vi "PicoScope4000Open.vi"(1 "Serial Number":string, 2 "Mode":u16(ring) items=["Dialog On Error", "no dialog - CloseUnit and Stop", "no dialog - Continue", "no dialog - Stop"], 5 "Use Serial Number":bool, 11 "error in (no error)":errorcluster) -> (4 "handle":i16, 12 "Max ADC value":i16, 14 "Unit Info":T1, 15 "error out":errorcluster)   [LabVIEW 2010]
doc: "This VI opens a PicoScope 4000 series and returns a handle to the device."
uses:
  ps4000.dll
panel:
  out "Pico 4000 Units":string
  out "serialLth":i16
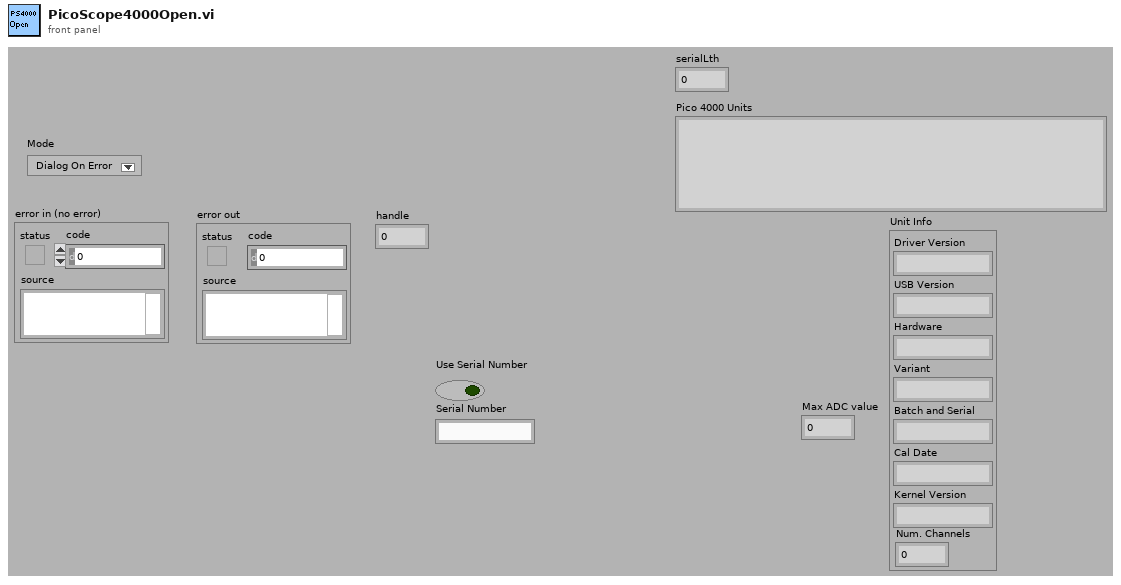
[diagram p1: front panel]
types:
  T1 = cluster{"Driver Version":string, "USB Version":string, "Hardware":string, "Variant":string, "Batch and Serial":string, "Cal Date":string, "Kernel Version":string, "Num. Channels":i16}
  T2 = cluster{"status":bool, "code":u32, "source":string}
  T3 = cluster{"Driver Version":string, "USB Version":string, "Hardware":string, "Variant":string, "Batch and Serial":string, "Cal Date":string, "Kernel Version":string}
  T4 = cluster{"Driver Version":string, "USB Version":string, "Hardware":string, "Variant":string, "Batch and Serial":string, "Cal Date":string, "Kernel Version":string, i16}
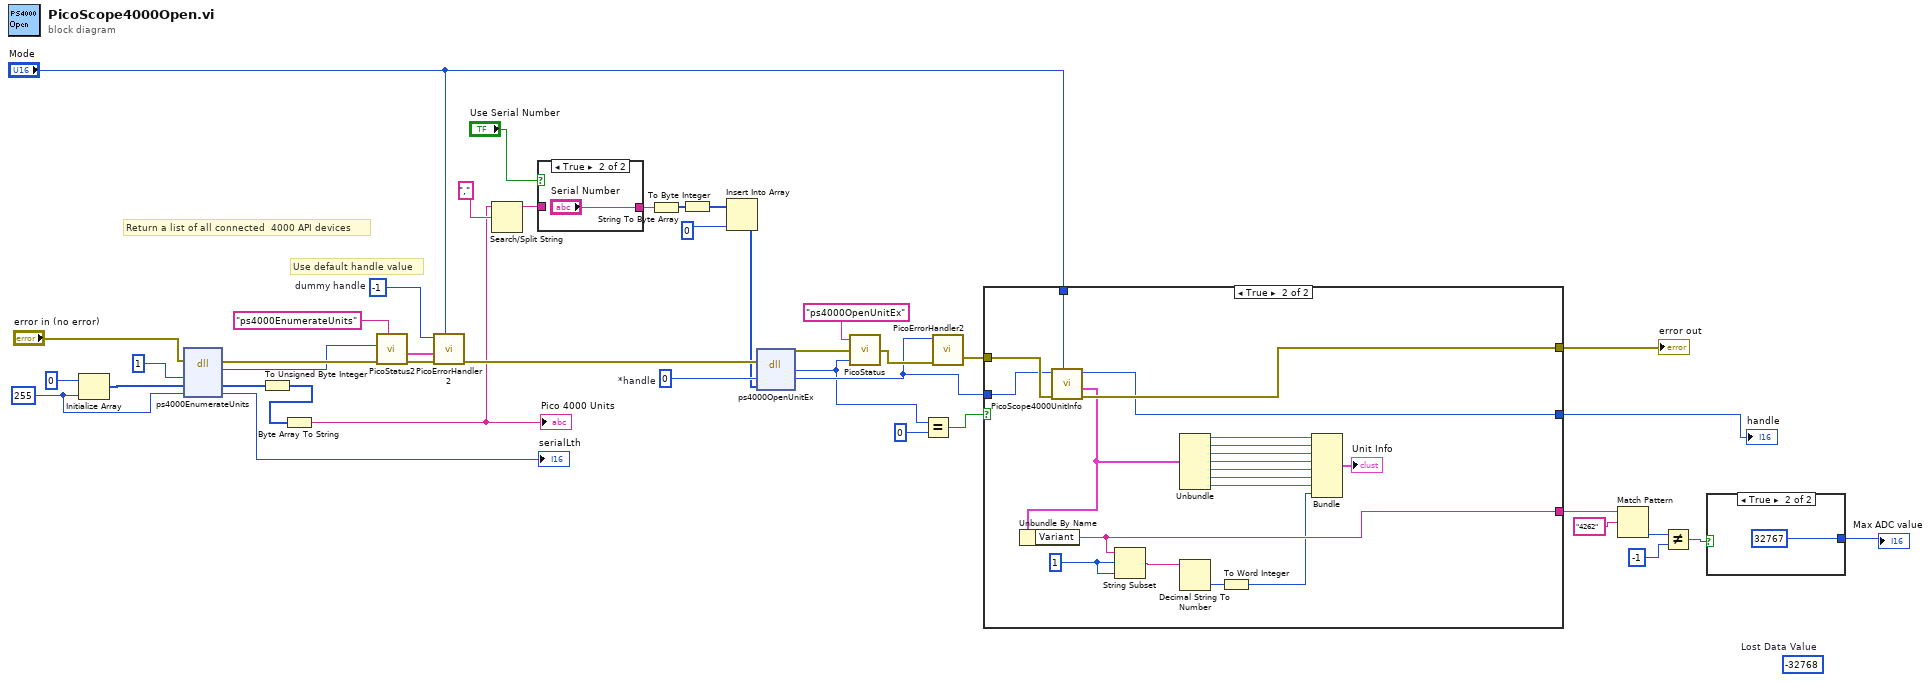
[diagram p0: block diagram]
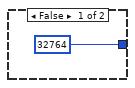
[diagram p3: hidden frame]
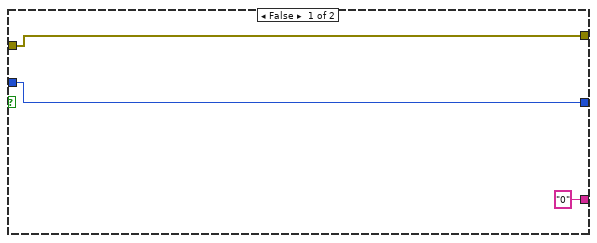
[diagram p4: hidden frame]
diagram:
  w17 = i16 -1  # dummy handle
  w20 = i16 255 ("dimension size")
  (unwired) i16 -32768  # Lost Data Value
  w33 = i16 0  # *handle
  # "Use default handle value"
  # "Return a list of all connected  4000 API devices"
  n1 = Initialize Array(i8 0 ("U8"), w20) -> (w22:i8[])
  n2 = dll-call lib="ps4000.dll" fn="ps4000EnumerateUnits"(error in="error in (no error)", "count"=i16 1, "serials"=w22, "serialLth"=w20) -> (error out=w5:errorcluster, "PICO_STATUS"=w4:u32, "serials"=w18:i8[], "serialLth"=→"serialLth":i16)  [unwired: 3 in, 1 out]
  n3 = To Unsigned Byte Integer(number=w18) -> (unsigned 8bit integer=w19:u8[])
  n4 = Byte Array To String(unsigned byte array=w19) -> (string=w9:string)
  "Pico 4000 Units" <- w9
  n5 = call "PicoStatus2.vi"("PICO source"="ps4000EnumerateUnits" ("source"), "Error in"=w5, "PICO STATUS"=w4) -> ("error out"=w7:errorcluster, "PICO_STATUS out"=w6:T2)  [unwired: 5 in]
  n6 = call "PicoErrorHandler2.vi"("Mode"="Mode", "error in (no error)"=w7, "PICO_STATUS in"=w6, "handle In"=w17) -> ("error out"=w32:errorcluster)  [unwired: 7 in]
  n7 = Search/Split String(string=w9, search string/char (-)=",") -> (substring before match=w15:string)  [unwired: 1 in, 2 out]
  n8 = case shown="True" "Use Serial Number" {
    tunnel: w15 -> [w43 _]
    tunnel: [w43 "Serial Number"] -> w11
    frame False {
    }
    frame True {
    }
  }
  n9 = String To Byte Array(string=w11) -> (unsigned byte array=w13:u8[])
  n10 = To Byte Integer(number=w13) -> (8bit integer=w14:i8[])
  n11 = Insert Into Array(array=w14, new element=i8 0 ("new element/subarray")) -> (w10:i8[])  [unwired: 1 in]
  n12 = dll-call lib="ps4000.dll" fn="ps4000OpenUnitEx"(error in=w32, "handle"=w33, "serial"=w10) -> (error out=w31:errorcluster, "PICO_STATUS"=w28:u32, "handle"=w29:i16)  [unwired: 3 in, 1 out]
  n13 = call "PicoStatus.vi"("PICO STATUS"=w28, "error in"=w31, "source"="ps4000OpenUnitEx") -> ("error out"=w39:errorcluster)
  n14 = Equal?(x=w28, y=i16 0) -> (x = y?=w42:bool)
  n15 = call "PicoErrorHandler2.vi"("error in (no error)"=w39, "handle In"=w29) -> ("error out"=w30:errorcluster)  [unwired: 9 in]
  n16 = case shown="True" w42 {
    tunnel: w29 -> [w47 w55]
    tunnel: [w47 w57] -> w25
    tunnel: [w46 w59] -> w1
    tunnel: w30 -> [w46 w56]
    tunnel: ["0" ("Variant") w50] -> w38
    tunnel: "Mode" -> [_ w48]
    frame False {
    }
    frame True {
      w51 = 1 ("offset (0)")
      n17 = call "PicoScope4000UnitInfo.vi"("Mode"=w48, "error in (no error)"=w56, "handle in"=w55) -> ("error out"=w59:errorcluster, "Unit Info"=w58:T3, "handle out"=w57:i16)  [unwired: 5 in, 1 out]
      n18 = Unbundle By Name(w58) -> ("Variant"=w50:string)
      n19 = String Subset(string=w50, offset (0)=w51, length (rest)=w51) -> (substring=w52:string)
      n20 = Unbundle(w58) -> ("Driver Version"=w66:string, "USB Version"=w65:string, "Hardware"=w64:string, "Variant"=w63:string, "Batch and Serial"=w62:string, "Cal Date"=w61:string, "Kernel Version"=w60:string)
      n21 = Decimal String To Number(string=w52) -> (number=w53:i32)  [unwired: 2 in, 1 out]
      n22 = To Word Integer(number=w53) -> (16bit integer=w49:i16)
      n23 = Bundle("Driver Version"=w66, "USB Version"=w65, "Hardware"=w64, "Variant"=w63, "Batch and Serial"=w62, "Cal Date"=w61, "Kernel Version"=w60, w49) -> (→"Unit Info":T4)  [unwired: 1 in]
    }
  }
  "handle" <- w25
  "error out" <- w1
  n24 = Match Pattern(string=w38, regular expression="4262") -> (offset past match=w36:i32)  [unwired: 1 in, 3 out]
  n25 = Not Equal?(x=w36, y=-1) -> (x != y?=w27:bool)
  n26 = case shown="True" w27 {
    tunnel: [i16 32764 ("Max ADC value") i16 32767 ("Max ADC value")] -> w26
    frame False {
    }
    frame True {
    }
  }
  "Max ADC value" <- w26
